vi "Test_Editor.vi"(8 "error in (no error)":errorcluster={"status"=FALSE, "code"=0, "source"="\"\""}, 10 "list of groups":string, 11 "TestDefinition":string) -> (0 "error out":errorcluster={"status"=FALSE, "code"=0, "source"="\"\""}, 2 "status ok":bool, 3 "Updated TestDefinition":string)   [LabVIEW 2026]
doc: "INTENT: Define tests and attached procedures. LOGIC: Edit prerequisite tests, repeat count, selected fault and shutdown sequence IDs, result rules."
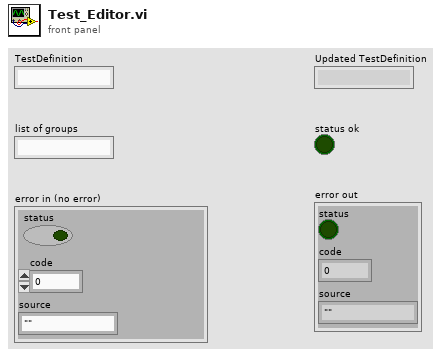
[diagram p1: front panel]
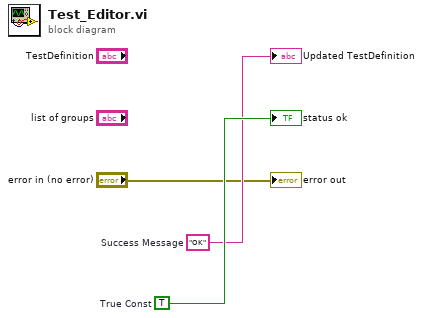
[diagram p0: block diagram]
diagram:
  w3 = TRUE  # True Const
  w2 = "OK"  # Success Message
  "Updated TestDefinition" <- w2
  "status ok" <- w3
  "error out" <- "error in (no error)"
